vi "Write Is Signed (I16)_.vi"(8 "error in (no error)":errorcluster, 10 "Is Signed (I16)?":bool=TRUE, 11 "Modbus_AO in":refnum<class "Modbus_AO.lvclass">) -> (0 "error out":errorcluster, 3 "Modbus_AO out":refnum<class "Modbus_AO.lvclass">)   [LabVIEW 2021, in "Modbus_AO.lvclass"]
uses:
  Modbus_AO.lvclass
  Modbus_AO.lvclass/Modbus_AO.ctl
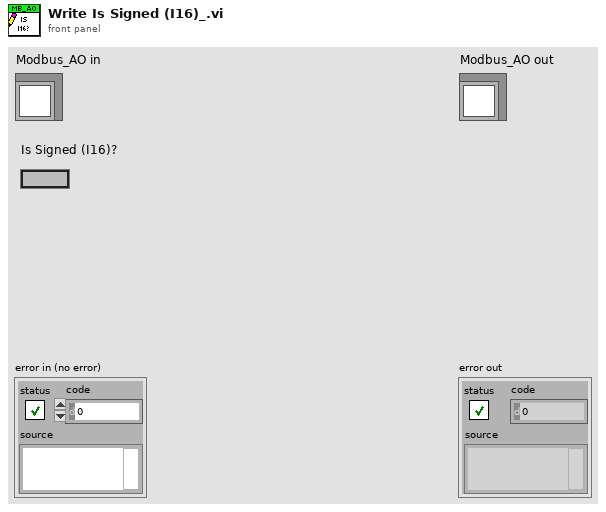
[diagram p1: front panel]
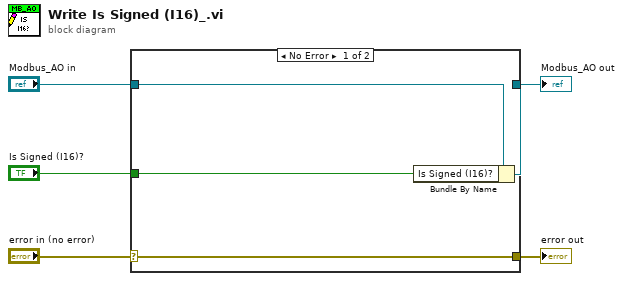
[diagram p0: block diagram]
diagram:
  n1 = case shown="No Error" "error in (no error)" {
    selector: "error in (no error)" -> [w9 w10]
    tunnel: [w9 w10] -> w4
    tunnel: [w7 w11] -> w2
    tunnel: "Modbus_AO in" -> [w8 w11]
    tunnel: "Is Signed (I16)?" -> [w6 _]
    frame No Error {
      n2 = Bundle By Name(cluster=w8, "Is Signed (I16)?"=w6) -> (w7:refnum<class "Modbus_AO.lvclass">)
    }
    frame Error {
    }
  }
  "error out" <- w4
  "Modbus_AO out" <- w2
